vi "Build Spec CLI.vi"(11 "Command line args":string[](array[string])) -> (2 "Output":string, 3 "Return code":i32)   [LabVIEW 2020]
doc: "Builds one build specification of a project for NI's LabVIEW CLI (RunVI): Command line args holds the project path and the build specification's name (target My Computer). Output lists the generated files, one per line, or the error; Return code is 0 on success, else the error code. tools\\build-package.ps1 runs it with LabVIEWCLI -OperationName RunVI because the CLI's own ExecuteBuildSpec operation, installed with a newer LabVIEW, does not load in LabVIEW 2020 (error 1498). Its connector pane is the one RunVI expects (pattern 4815, Command line args at 11, Output at 2, Return code at 3)."
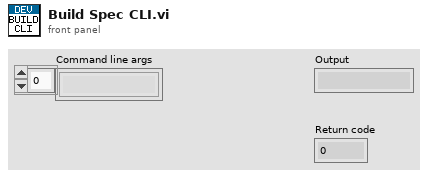
[diagram p1: front panel]
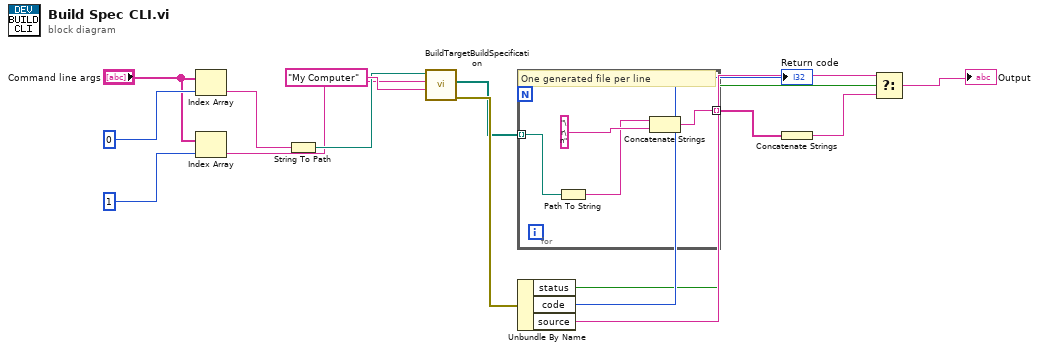
[diagram p0: block diagram]
diagram:
  n1 = Index Array(array="Command line args", index=0) -> (element=w4:string)
  n2 = Index Array(array="Command line args", index=1) -> (element=w5:string)
  n3 = String To Path(string=w4) -> (path=w6:path)
  n4 = call <vilib>:"BuildTargetBuildSpecification.vi"("Name of target (My Computer)"="My Computer", "Name of build specification (if empty: build all)"=w5, "Path to project"=w6) -> ("error out"=w9:errorcluster, "Generated files"=w8:path[])  [unwired: 7 in]
  n5 = for {
    tunnel: w8 -> [w16] mode=indexing
    tunnel: [w19] -> w10 mode=indexing
    # "One generated file per line"
    n6 = Path To String(path=w16) -> (string=w17:string)
    n7 = Concatenate Strings(w17, "\r\n") -> (w19:string)
  }
  n8 = Unbundle By Name(w9) -> ("status"=w12:bool, "code"=→"Return code":i32, "source"=w14:string)
  n9 = Concatenate Strings(w10) -> (w11:string)
  n10 = Select(t=w14, s=w12, f=w11) -> (s? t:f=→"Output":string)
